vi "Initialize.vi"(8 "error in":errorcluster, 11 "Plugin in":refnum<class "NVH Condition Indicators.lvclass">) -> (0 "error out":errorcluster, 3 "Plugin out":refnum<class "NVH Condition Indicators.lvclass">)   [LabVIEW 2026, in "NVH Condition Indicators.lvlib" / "NVH Condition Indicators.lvclass"]
uses:
  NVH Condition Indicators.lvclass
  C:/Program Files/National Instruments/LabVIEW 2026/vi.lib/FlexLogger/SDK/PluginSDK.lvlibp/PEFClasses/SDK/Plugin/Plugin.lvclass
  <vilib>/FlexLogger/SDK/PluginSDK.lvlibp/PEFClasses/SDK/System Interface/Resampling Mode.ctl
  <vilib>/FlexLogger/SDK/PluginSDK.lvlibp/PEFClasses/SDK/Channel/Data Type_v2.ctl
  <vilib>/FlexLogger/SDK/PluginSDK.lvlibp/PEFClasses/SDK/Producer Channel/Producer Channel.lvclass
  C:/Program Files/National Instruments/LabVIEW 2026/vi.lib/FlexLogger/SDK/PluginSDK.lvlibp/PEFClasses/SDK/Channel/Channel.lvclass
  <vilib>/FlexLogger/SDK/PluginSDK.lvlibp/PEFClasses/SDK/Plugin/ParameterAccess/Write Single Channel.vi
  <vilib>/FlexLogger/SDK/PluginSDK.lvlibp/PEFClasses/SDK/Plugin/ParameterAccess/Write Enum.vi
  <vilib>/FlexLogger/SDK/PluginSDK.lvlibp/PEFClasses/SDK/Producer Channel/Create Producer Channel_v2.vi
  <vilib>/FlexLogger/SDK/PluginSDK.lvlibp/PEFClasses/SDK/Plugin/Plugin.lvclass
  C:/Program Files/National Instruments/LabVIEW 2026/vi.lib/FlexLogger/SDK/PluginSDK.lvlibp/PEFClasses/SDK/Processing Element/Processing Element.lvclass
  C:/Users/dihidalg/Documents/GIT/Demos/SnV-Flexlogger-Plugin-PoC/src/FlexLogger-Plugin/NVH Condition Indicators/NVH Condition Indicators.lvclass
  <vilib>/FlexLogger/SDK/PluginSDK.lvlibp/PEFClasses/SDK/System Interface/System Interface.lvclass
  <vilib>/FlexLogger/SDK/PluginSDK.lvlibp
  <vilib>/FlexLogger/SDK/PluginSDK.lvlibp/PEFClasses/SDK/Channel/Channel.lvclass
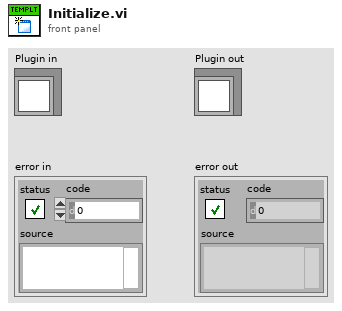
[diagram p1: front panel]
types:
  T1 = typedef "PluginSDK.lvlibp/System Interface.lvclass/Resampling Mode.ctl" = enum16{"No Resampling", "Custom Rate", "Maximum Rate", "Minimum Rate"}
  T2 = typedef "PluginSDK.lvlibp/Channel.lvclass/Data Type_v2.ctl" = u16
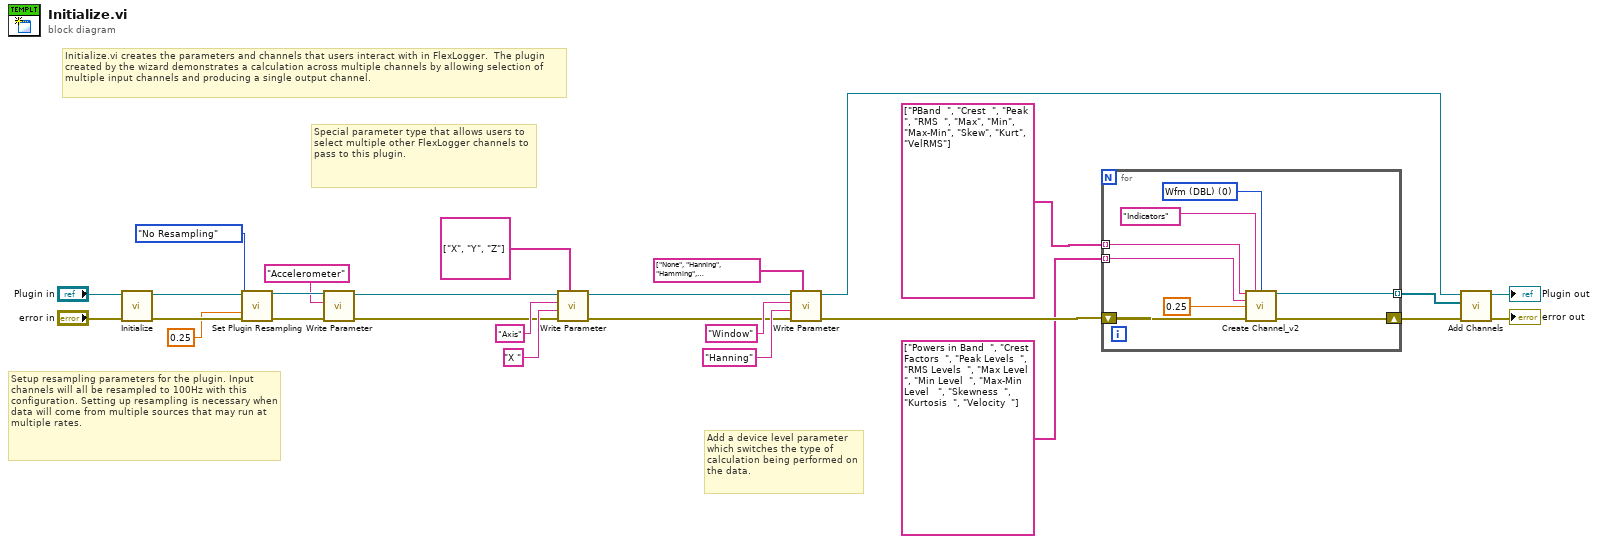
[diagram p0: block diagram]
diagram:
  # "Add a device level parameter which switches the type of calculation being performed on the data."
  # "Setup resampling parameters for the plugin. Input channels will all be resampled to 100Hz with this configuration. Setting up resampling is necessary when data will come from multiple sources that may run at multiple rates."
  # "Special parameter type that allows users to select multiple other FlexLogger channels to pass to this plugin."
  # "Initialize.vi creates the parameters and channels that users interact with in FlexLogger.  The plugin created by the wizard demonstrates a calculation across multiple channels by allowing selection of multiple input channels and producing a single output channel."
  n1 = call-parent "Initialize.vi"("error in (no error)"="error in", "Plugin in"="Plugin in") -> ("error out"=w23:errorcluster, "Plugin out"=w24:refnum<class "NVH Condition Indicators.lvclass">)  [unwired: 8 in]
  n2 = call <vilib>:"Set Plugin Resampling.vi"("Plugin in"=w24, "Resampling Mode"=Resampling_Mode."No Resampling", "Block Size (s)"=0.25, "error in (no error)"=w23) -> ("Plugin out"=w11:refnum<class "NVH Condition Indicators.lvclass">, "error out"=w10:errorcluster)  [unwired: 10 in]
  n3 = call-poly <vilib>:"Write Parameter.vi"("error in (no error)"=w10, "Name (Unique Channel Identifier)"="Accelerometer" ("String"), "Plugin in"=w11) -> ("error out"=w3:errorcluster, "Plugin out"=w5:refnum<class "NVH Condition Indicators.lvclass">)  [unwired: 7 in]
  n4 = call-poly <vilib>:"Write Parameter.vi"("Possible Values"=string[] ["X", "Y", "Z"], "error in (no error)"=w3, "Current Value"="X ", "Name"="Axis", "Plugin in"=w5) -> ("error out"=w2:errorcluster, "Plugin out"=w4:refnum<class "NVH Condition Indicators.lvclass">)  [unwired: 5 in]
  n5 = call-poly <vilib>:"Write Parameter.vi"("Possible Values"=string[] ["None", "Hanning", "Hamming", "Blackman-Harris", "Exact Blackman", "Blackman", "Flat Top", "4 Term B-Harris ", "7 Term B-Harris", "Low Sidelobe", "Force", "Exponential", "Blackman Nuttall", "Triangle", "Bartlett-Hanning", "Bohman", "Parzen", "Welch", "Kaiser", "Dolph-Chebyshev", "Gaussian"] ("Strings []"), "error in (no error)"=w2, "Current Value"="Hanning", "Name"="Window", "Plugin in"=w4) -> ("error out"=w16:errorcluster, "Plugin out"=w14:refnum<class "NVH Condition Indicators.lvclass">)  [unwired: 5 in]
  n6 = for {
    tunnel: [w32] -> w12 mode=indexing
    tunnel: string[] ["PBand  ", "Crest  ", "Peak  ", "RMS  ", "Max", "Min", "Max-Min", "Skew", "Kurt", "VelRMS"] ("Possible Values") -> [w28] mode=indexing
    shift-right: [w35] -> w22
    shift-left: w16 -> [w34]
    tunnel: string[] ["Powers in Band  ", "Crest Factors  ", "Peak Levels  ", "RMS Levels  ", "Max Level  ", "Min Level  ", "Max-Min Level   ", "Skewness  ", "Kurtosis  ", "Velocity  "] ("Possible Values") -> [w29] mode=indexing
    w33 = T2 0 items=["Wfm (DBL)", "Wfm (Digital)", "String"] ("Data Type")
    n7 = call-poly <vilib>:"Create Channel_v2.vi"("Unique Channel Identifier"=w28, "Display Group"="Indicators" ("String"), "Data Type"=w33, "Default Channel Name"=w29, "dt(sec)"=0.25, "error in (no error)"=w34) -> ("Producer Channel"=w32:refnum<class "Producer Channel.lvclass">, "error out"=w35:errorcluster)  [unwired: 8 in]
  }
  n8 = call <vilib>:"Add Channels.vi"("error in (no error)"=w22, "Channels"=w12, "Plugin in"=w14) -> ("error out"=→"error out":errorcluster, "Plugin out"=→"Plugin out":refnum<class "NVH Condition Indicators.lvclass">)  [unwired: 7 in]
